vi "VHist - Interpolate DBL History.vi"(6 "method (linear)":T1(ring), 8 "error in":errorcluster, 9 "time stamp (0: now)":dbl format="%<%H:%M:%S%2u\n%d/%m/%Y>T", 10 "history data":dbl[](array[numeric]) format="%.2f", 11 "time stamps":dbl[](array[numeric]) format="%<%H:%M:%S%2u\n%d/%m/%Y>T") -> (0 "error out":errorcluster, 2 "history data out":dbl[](array[numeric]) format="%.2f", 3 "time stamps out":dbl[](array[numeric]) format="%<%H:%M:%S%2u\n%d/%m/%Y>T")   [LabVIEW 2021]
doc: "The VI inserts the specified timestamp and either interpolated or extrapolated value at this timestamp into an appropriate position in DBL history. Interpolation method can be linear (by default), spline, polynominal or rational.\n\n::: CalcExpress Toolkit :::\nCopyright (c) 2000-2026 Konstantin Shifershteyn. All rights reserved."
uses:
  <vilib>/Analysis/NI_AALPro.lvlib
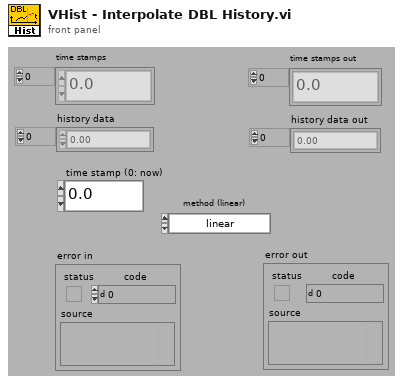
[diagram p1: front panel]
types:
  T1 = enum16{"linear", "spline", "polynominal", "rational"}
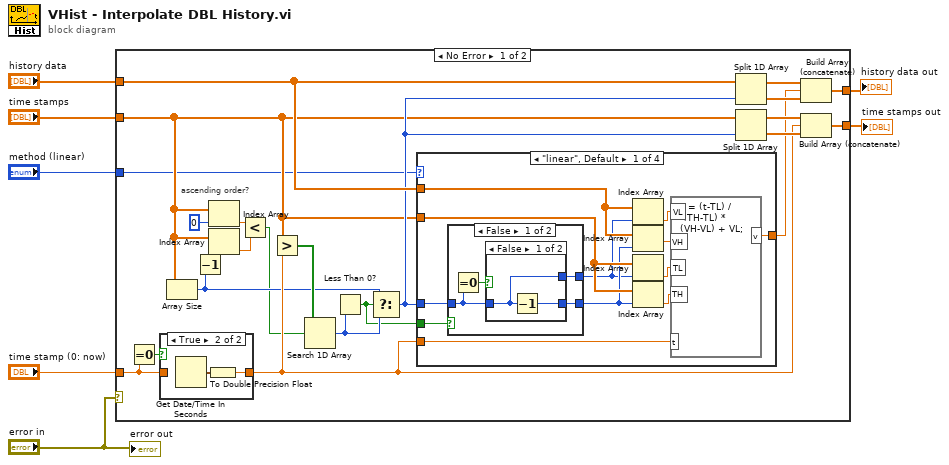
[diagram p0: block diagram]
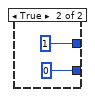
[diagram p2: hidden frame]
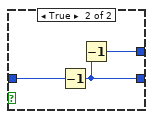
[diagram p3: hidden frame]
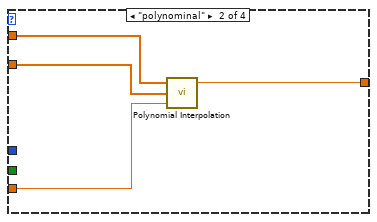
[diagram p4: hidden frame]
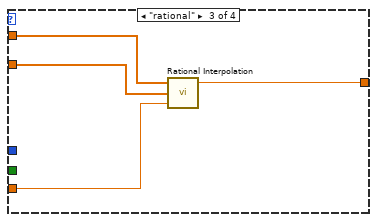
[diagram p5: hidden frame]
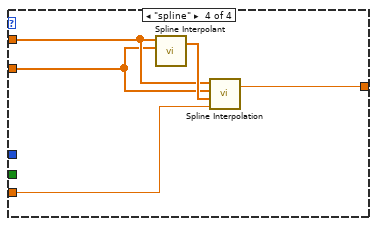
[diagram p6: hidden frame]
diagram:
  n1 = case shown="No Error" "error in" {
    tunnel: "history data" -> [w29 w71]
    tunnel: [w24 w70] -> w6
    tunnel: [w23 w71] -> w5
    tunnel: "time stamps" -> [w11 w70]
    tunnel: "time stamp (0: now)" -> [w16 _]
    tunnel: "method (linear)" -> [w8 _]
    frame No Error {
      # "ascending order?"
      n2 = Equal To 0?(x=w16) -> (x = 0?=w30:bool)
      n3 = case shown="True" w30 {
        tunnel: [w67 w69] -> w20
        tunnel: w16 -> [w67 _]
        frame False {
        }
        frame True {
          n4 = Get Date/Time In Seconds() -> (seconds since 1Jan1904=w68:timestamp)
          n5 = To Double Precision Float(number=w68) -> (double precision float=w69:dbl)
        }
      }
      n6 = Array Size(array=w11) -> (size(s)=w10:i32)
      n7 = Decrement(x=w10) -> (x-1=w12:i32)
      n8 = Index Array(array=w11, index=0) -> (element=w14:dbl)
      n9 = Index Array(array=w11, index=w12) -> (element=w13:dbl)
      n10 = Less?(x=w14, y=w13) -> (x < y?=w9:bool)
      n11 = Greater?(x=w11, y=w20) -> (0:w21:bool[])
      n12 = Search 1D Array(1D array=w21, element=w9) -> (index of element=w19:i32)  [unwired: 1 in]
      n13 = Less Than 0?(x=w19) -> (x < 0?=w18:bool)
      n14 = Select(t=w10, s=w18, f=w19) -> (s? t:f=w17:i32)
      n15 = case shown="\"linear\", Default" w8 {
        tunnel: w11 -> [w40 w57 w60 w63]
        tunnel: w20 -> [w42 w56 w59 w65]
        tunnel: w29 -> [w35 w55 w61 w64]
        tunnel: [w41 w54 w58 w62] -> w22
        tunnel: w18 -> [w34 _ _ _]
        tunnel: w17 -> [w33 _ _ _]
        frame "linear", Default {
          n16 = case shown="False" w34 {
            tunnel: w33 -> [w43 w53]
            tunnel: [w46 w52] -> w32
            tunnel: [w45 w51] -> w31
            frame False {
              n17 = Equal To 0?(x=w43) -> (x = 0?=w44:bool)
              n18 = case shown="False" w44 {
                tunnel: [w47 0] -> w46
                tunnel: [w48 1] -> w45
                tunnel: w43 -> [w48 _]
                frame False {
                  n19 = Decrement(x=w48) -> (x-1=w47:i32)
                }
                frame True {
                }
              }
            }
            frame True {
              n20 = Decrement(x=w53) -> (x-1=w52:i32)
              n21 = Decrement(x=w52) -> (x-1=w51:i32)
            }
          }
          n22 = Index Array(array=w35, index=w31) -> (element=w39:dbl)
          n23 = Index Array(array=w35, index=w32) -> (element=w38:dbl)
          n24 = Index Array(array=w40, index=w31) -> (element=w37:dbl)
          n25 = Index Array(array=w40, index=w32) -> (element=w36:dbl)
          n26 = formula code="v = (t-TL) /\n (TH-TL) * \n(VH-VL) + VL;"("TH"=w36, "TL"=w37, "VH"=w38, "VL"=w39, "t"=w42) -> ("v"=w41:dbl)
        }
        frame "polynominal" {
          n27 = call <vilib>:"Polynomial Interpolation.vi"("x value"=w56, "X"=w57, "Y"=w55) -> ("interpolation value"=w54:dbl)  [unwired: 2 out]
        }
        frame "rational" {
          n28 = call <vilib>:"Rational Interpolation.vi"("x value"=w59, "X"=w60, "Y"=w61) -> ("interpolation value"=w58:dbl)  [unwired: 2 out]
        }
        frame "spline" {
          n29 = call <vilib>:"Spline Interpolant.vi"("X"=w63, "Y"=w64) -> ("Interpolant"=w66:dbl[])  [unwired: 2 in, 1 out]
          n30 = call <vilib>:"Spline Interpolation.vi"("x value"=w65, "Interpolant"=w66, "X"=w63, "Y"=w64) -> ("interpolation value"=w62:dbl)  [unwired: 1 out]
        }
      }
      n31 = Split 1D Array(array=w29, index=w17) -> (first subarray=w28:dbl[], second subarray=w27:dbl[])
      n32 = Split 1D Array(array=w11, index=w17) -> (first subarray=w26:dbl[], second subarray=w25:dbl[])
      n33 = Build Array (concatenate)(w28, w22, w27) -> (w23:dbl[])
      n34 = Build Array (concatenate)(w26, w20, w25) -> (w24:dbl[])
    }
    frame Error {
    }
  }
  "time stamps out" <- w6
  "history data out" <- w5
  "error out" <- "error in"
